vi "basic-lifetime-test.vi"(8 "error in (no error)":errorcluster) -> (0 "error out":errorcluster)   [LabVIEW 2013]
uses:
  src/SMO/SMO.lvclass
  src/SMO/Typedefs/SMOState --Enum.ctl
  <vilib>/addons/_JKI Toolkits/Caraya/classes/Test/Test.lvclass
  <vilib>/addons/_JKI Toolkits/Caraya/classes/Assert/Assert.lvclass
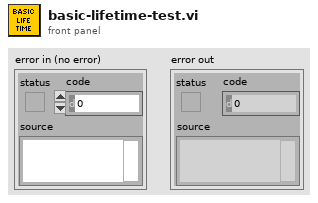
[diagram p1: front panel]
types:
  T1 = typedef "SMO.lvclass/SMOState --Enum.ctl" = enum16{"unknown", "Created", "Started", "Stopped"}
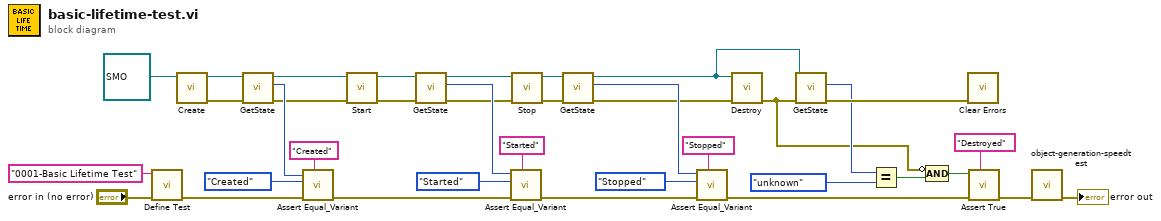
[diagram p0: block diagram]
diagram:
  n1 = call <vilib>:"Define Test.vi"("error in (no error)"="error in (no error)", "Label (VI Title)"="0001-Basic Lifetime Test") -> ("error out"=w32:errorcluster)  [unwired: 9 in]
  n2 = call "Create.vi"("SMO"=refnum<class "SMO.lvclass"> refnum ("SMO.lvclass")) -> ("error out"=w33:errorcluster, "SMO out"=w36:refnum<class "SMO.lvclass">)  [unwired: 8 in, 1 out]
  n3 = call "GetState.vi"("error in (no error)"=w33, "SMO"=w36) -> ("error out"=w28:errorcluster, "SMO State"=w31:T1, "SMO out"=w35:refnum<class "SMO.lvclass">)  [unwired: 7 in]
  n4 = call <vilib>:"Assert Equal_Variant.vi"("Label"="Created" ("Label (VI Title)"), "error in (no error)"=w32, "Y"=SMOState_--Enum."Created" ("SMO State"), "X"=w31) -> ("error out"=w24:errorcluster)  [unwired: 7 in]
  n5 = call "Start.vi"("error in (no error)"=w28, "SMO"=w35) -> ("error out"=w26:errorcluster, "SMO out"=w27:refnum<class "SMO.lvclass">)  [unwired: 8 in]
  n6 = call "GetState.vi"("error in (no error)"=w26, "SMO"=w27) -> ("error out"=w20:errorcluster, "SMO State"=w22:T1, "SMO out"=w21:refnum<class "SMO.lvclass">)  [unwired: 7 in]
  n7 = call <vilib>:"Assert Equal_Variant.vi"("Label"="Started" ("Label (VI Title)"), "error in (no error)"=w24, "Y"=SMOState_--Enum."Started" ("SMO State"), "X"=w22) -> ("error out"=w14:errorcluster)  [unwired: 7 in]
  n8 = call "Stop.vi"("error in (no error)"=w20, "SMO"=w21) -> ("error out"=w17:errorcluster, "SMO out"=w16:refnum<class "SMO.lvclass">)  [unwired: 8 in]
  n9 = call "GetState.vi"("error in (no error)"=w17, "SMO"=w16) -> ("error out"=w13:errorcluster, "SMO State"=w15:T1, "SMO out"=w12:refnum<class "SMO.lvclass">)  [unwired: 7 in]
  n10 = call <vilib>:"Assert Equal_Variant.vi"("Label"="Stopped" ("Label (VI Title)"), "error in (no error)"=w14, "Y"=SMOState_--Enum."Stopped" ("SMO State"), "X"=w15) -> ("error out"=w5:errorcluster)  [unwired: 7 in]
  n11 = call "Destroy.vi"("error in (no error)"=w13, "SMO"=w12) -> ("error out"=w6:errorcluster)  [unwired: 9 in]
  n12 = call "GetState.vi"("error in (no error)"=w6, "SMO"=w12) -> ("error out"=w10:errorcluster, "SMO State"=w8:T1)  [unwired: 7 in, 1 out]
  n13 = Equal?(x=w8, y=SMOState_--Enum."unknown" ("SMO State")) -> (x = y?=w7:bool)
  n14 = Compound Arithmetic op=AND(invert w6, w7) -> (w3:bool)
  n15 = call <vilib>:"Clear Errors.vi"("error in (no error)"=w10) -> ()  [unwired: 6 in, 1 out]
  n16 = call <vilib>:"Assert True.vi"("Label"="Destroyed" ("Label (VI Title)"), "error in (no error)"=w5, "True?"=w3) -> ("error out"=w2:errorcluster)  [unwired: 8 in]
  n17 = call "object-generation-speedtest.vi"("error in (no error)"=w2) -> ("error out"=→"error out":errorcluster)  [unwired: 10 in]
